vi "Luanch.vi"(9 "포트":u16=5025, 10 "문자열":string="127.0.0.1") -> ()   [LabVIEW 2023]
uses:
  Instrument Manager.lvclass
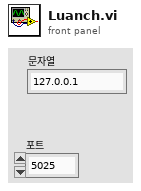
[diagram p1: front panel]
types:
  T1 = cluster{"Reader Q":refnum<queue>, "Writer Q":refnum<queue>}
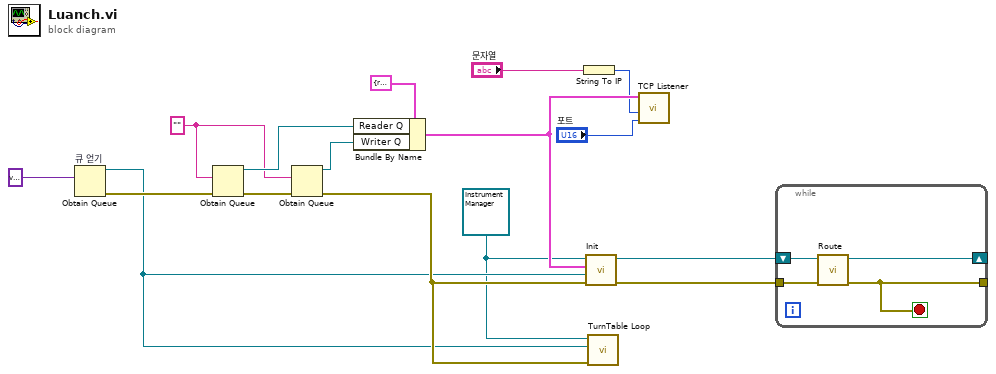
[diagram p0: block diagram]
diagram:
  w2 = refnum<class "Instrument Manager.lvclass"> refnum ("Instrument Manager 입력")
  w12 = ""
  n1 = Obtain Queue "큐 얻기"(element data type=variant) -> (queue out=w7:refnum<queue>, error out=w9:errorcluster)  [unwired: 4 in, 1 out]
  n2 = Obtain Queue(element data type=w12, error in (no error)=w9) -> (queue out=w14:refnum<queue>, error out=w16:errorcluster)  [unwired: 3 in, 1 out]
  n3 = Obtain Queue(element data type=w12, error in (no error)=w16) -> (queue out=w13:refnum<queue>, error out=w8:errorcluster)  [unwired: 3 in, 1 out]
  n4 = Bundle By Name(cluster=T1 {"Reader Q"=refnum, "Writer Q"=refnum} ("Queue Ref"), "Reader Q"=w14, "Writer Q"=w13) -> (w11:T1)
  n5 = String To IP(1:"문자열") -> (0:w3:u32)
  n6 = call "Init.vi"("error in (no error)"=w8, "Sad Queue"=w7, "Queue Ref"=w11, "Instrument Manager 입력"=w2) -> ("error out"=w6:errorcluster, "Instrument Manager 출력"=w5:refnum<class "Instrument Manager.lvclass">)  [unwired: 6 in]
  n7 = call "TurnTable Loop.vi"("error in (no error)"=w8, "Sad Queue"=w7, "Instrument Manager 입력"=w2) -> ()  [unwired: 7 in, 2 out]
  n8 = call "TCP Listener.vi"("포트"="포트", "네트워크 주소"=w3, "Queue Ref"=w11) -> ()  [unwired: 9 in]
  n9 = while {
    shift-right: [w17] -> _
    shift-left: w5 -> [w18]
    tunnel: w6 -> [w20]
    tunnel: [w19] -> _
    stop <- w19 stop-if-true
    n10 = call "Route.vi"("error in (no error)"=w20, "Instrument Manager 입력"=w18) -> ("error out"=w19:errorcluster, "Instrument Manager 출력"=w17:refnum<class "Instrument Manager.lvclass">)  [unwired: 8 in]
  }
